vi "Calculate Cubic Bezier Point.vi"(7 "t":dbl, 8 "d":dbl, 9 "c":dbl, 10 "b":dbl, 11 "a":dbl) -> (3 "f(t)":dbl)   [LabVIEW 2019, in "Tool Path.lvclass"]
uses:
  Tool Path.lvclass
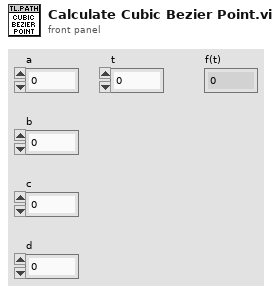
[diagram p1: front panel]
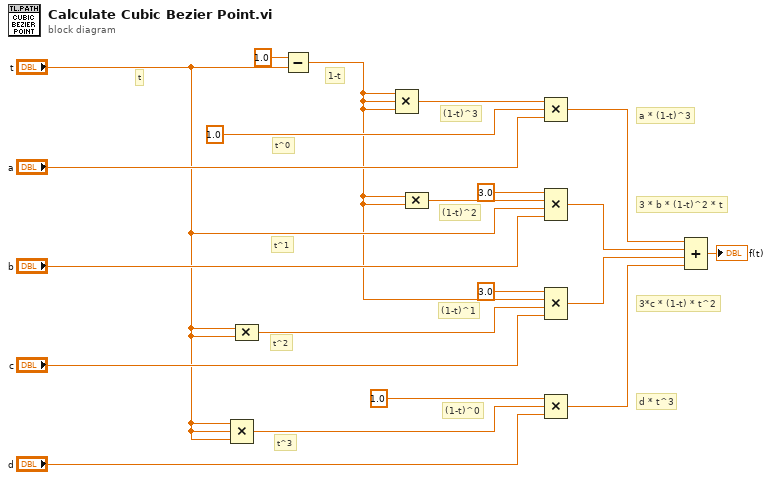
[diagram p0: block diagram]
diagram:
  # "t^3"
  # "t^2"
  # "t^1"
  # "t^0"
  # "(1-t)^0"
  # "(1-t)^1"
  # "(1-t)^2"
  # "(1-t)^3"
  # "1-t"
  # "d * t^3"
  # "3*c * (1-t) * t^2"
  # "3 * b * (1-t)^2 * t"
  # "a * (1-t)^3"
  # "t"
  n1 = Compound Arithmetic op=MULTIPLY("t", "t", "t") -> (w8:dbl)
  n2 = Compound Arithmetic op=MULTIPLY("t", "t") -> (w7:dbl)
  n3 = Subtract(x=1.0, y="t") -> (x-y=w1:dbl)
  n4 = Compound Arithmetic op=MULTIPLY(w1, w1, w1) -> (w2:dbl)
  n5 = Compound Arithmetic op=MULTIPLY(w1, w1) -> (w3:dbl)
  n6 = Compound Arithmetic op=MULTIPLY(w2, 1.0 ("y"), "a") -> (w13:dbl)
  n7 = Compound Arithmetic op=MULTIPLY(3.0 ("value"), w3, "t", "b") -> (w12:dbl)
  n8 = Compound Arithmetic op=MULTIPLY(3.0 ("value"), w1, w7, "c") -> (w11:dbl)
  n9 = Compound Arithmetic op=MULTIPLY(1.0 ("y"), w8, "d") -> (w10:dbl)
  n10 = Compound Arithmetic op=ADD(w13, w12, w11, w10) -> (→"f(t)":dbl)
